vi "Beer_Pong_obstacle.vi"(8 "error in (no error)":errorcluster, 11 "Tableau lidar":dbl[][](array[numeric])=[[0.0, 1.0, 2.0, 3.0, 4.0, 5.0, 6.0, 7.0, 8.0, 9.0, 10.0, 11.0, 12.0, 13.0, 14.0, 15.0, 16.0, 17.0, 18.0, 19.0, 20.0, 21.0, 22.0, 23.0, 24.0, 25.0, 26.0, 27.0, 28.0, 29.0, 30.0, 31.0, 32.0, 33.0, 34.0, 35.0], [20.0, 15.0, 30.0, 31.0, 42.0, 50.0, 51.0, 60.0, 20.0, 15.0, 30.0, 31.0, 42.0, 50.0, 51.0, 60.0, 20.0, 15.0, 30.0, 31.0, 42.0, 50.0, 51.0, 60.0, 20.0, 15.0, 30.0, 31.0, 42.0, 50.0, 51.0, 60.0, 20.0, 15.0, 30.0, 31.0], [0.0, 0.0, 0.0, 0.0, 0.0, 0.0, 0.0, 0.0, 0.0, 0.0, 0.0, 0.0, 0.0, 0.0, 0.0, 0.0, 0.0, 0.0, 0.0, 0.0, 0.0, 0.0, 0.0, 0.0, 0.0, 0.0, 0.0, 0.0, 0.0, 0.0, 0.0, 0.0, 0.0, 0.0, 0.0, 0.0]]) -> (0 "error out":errorcluster, 2 "Distance cible":dbl, 3 "Angle cible":dbl)   [LabVIEW 2017]
panel:
  out "Cibles Detectes":dbl[][](array[numeric])
  in  "Delta Distance (cm)":dbl=10.0
  in  "Delta Angle (°)":dbl=3.0
  out "Zone 3 Bis":dbl[][](array[numeric])
  out "Detec part 3":dbl[][](array[numeric])
  out "Nbr ° à enlever début 2":i32
  out "Nbr ° à enlever fin 2":i32
  out "Début detec 3":i32
  out "Detec part 4":dbl[][](array[numeric])
  out "Moitié de Alpha":dbl
  in  "Alpha":i32=180
  in  "L3":dbl=100.0
  out "Zone 3":dbl[][](array[numeric])
  out "Zone de detection":dbl[][](array[numeric])
  out "Nbr ° à enlever fin":dbl
  out "Début detec 2":dbl
  out "Detec part 2":dbl[][](array[numeric])
  out "Nbr ° à enlever début":dbl
  out "Detec part 1":dbl[][](array[numeric])
  out "Moitié de ZM":dbl
  in  "Angle zone morte (°)":i32=170
  out "Angles / distance / statut":dbl[][](array[numeric])
  # "Face Avant"
  # "Debug"
  # "Zone morte retirée"
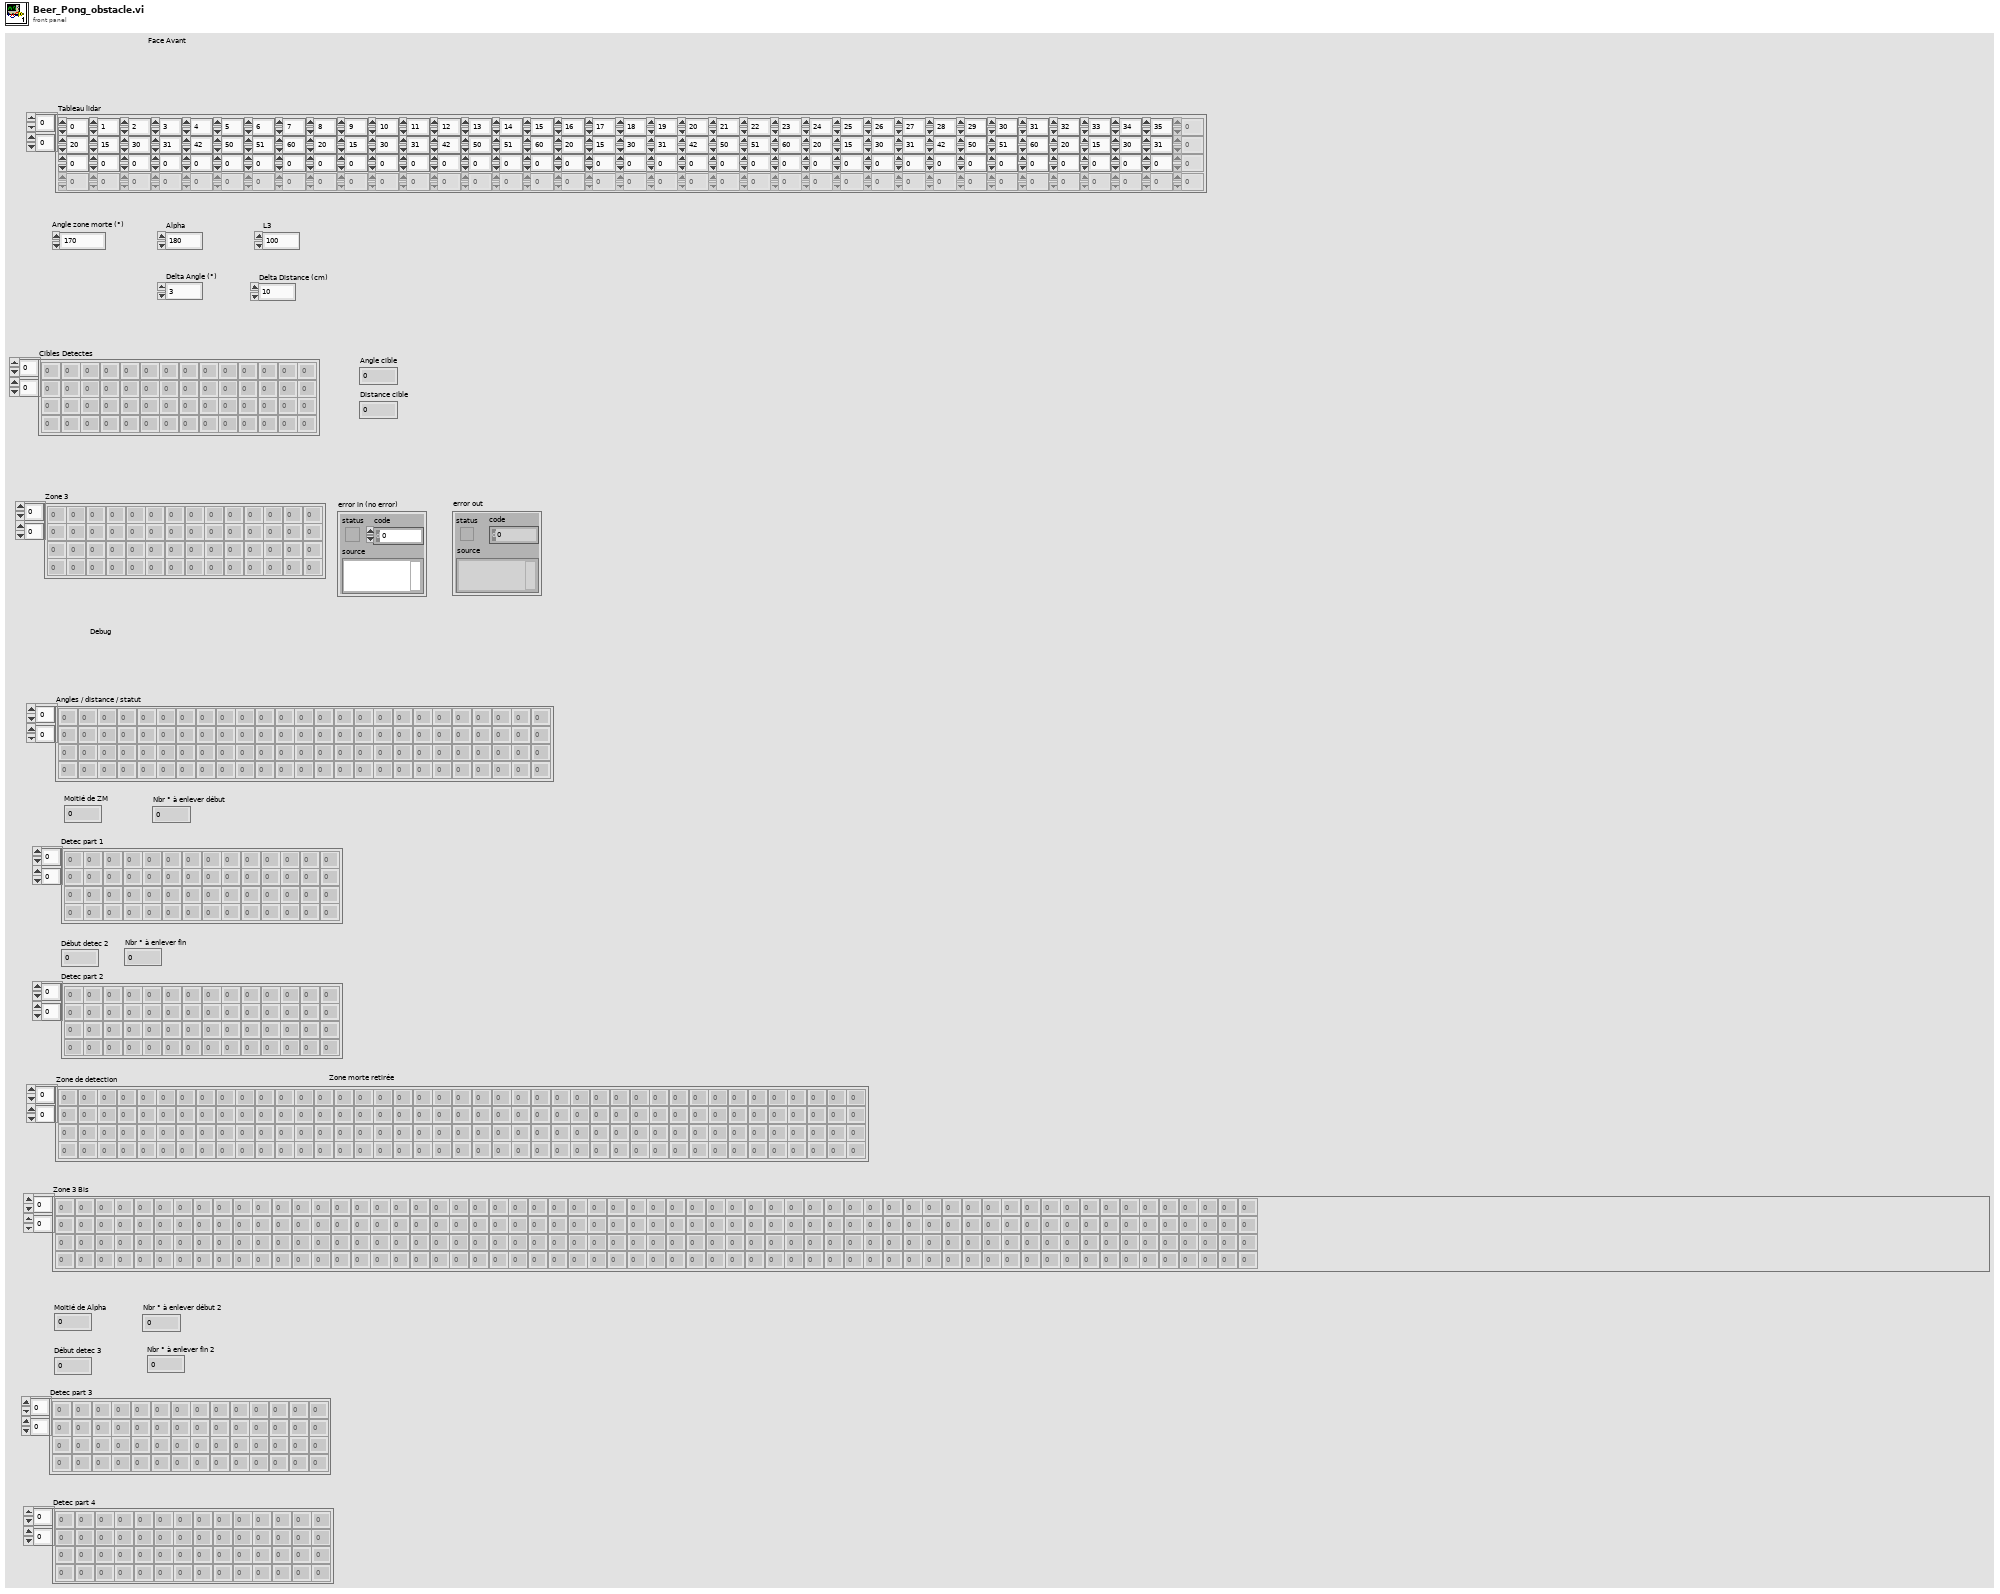
[diagram p1: front panel]
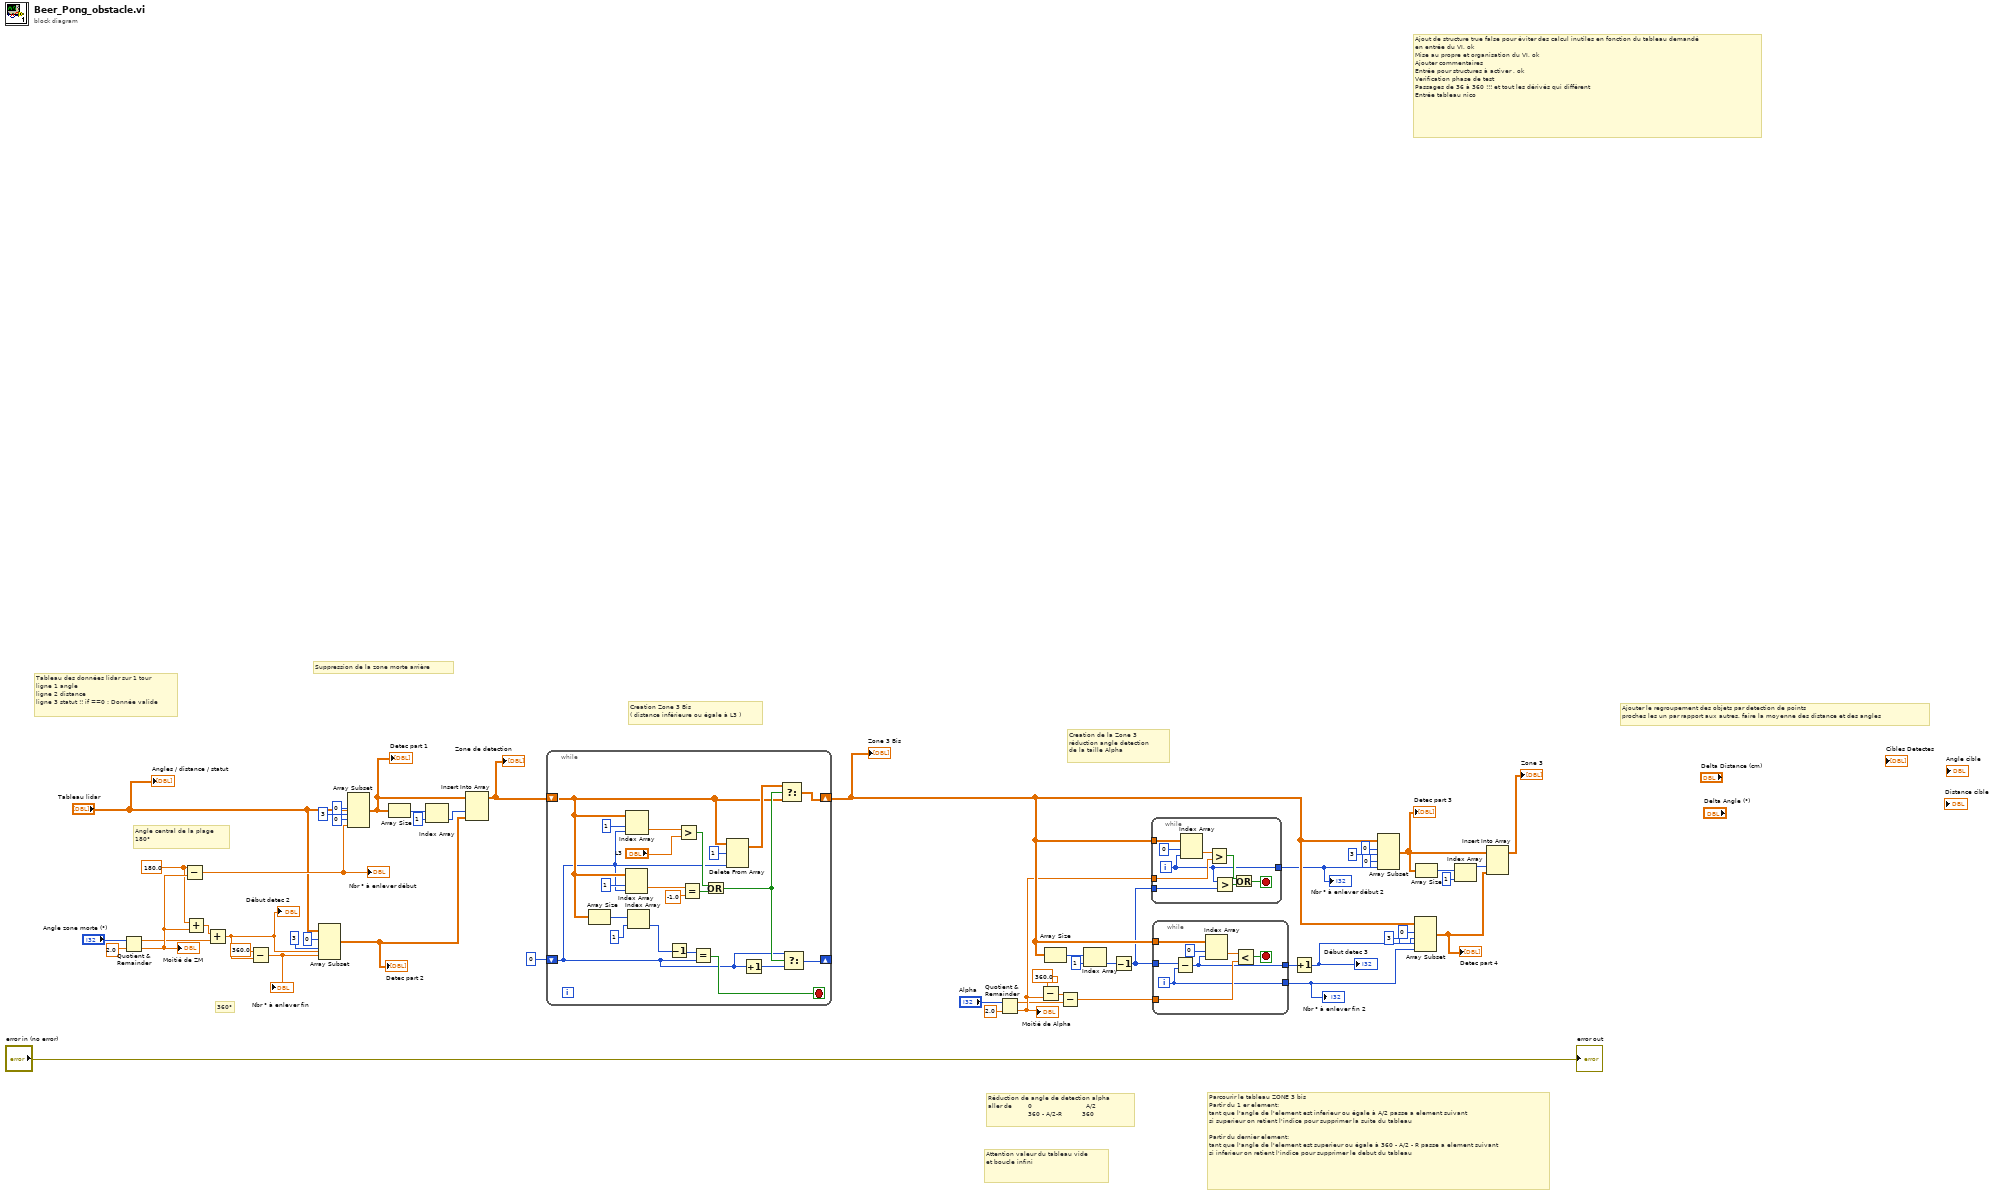
[diagram p0: block diagram]
diagram:
  w30 = 180.0 ("x")
  # "Ajouter le regroupement des objets par detection de points\nproches les un par rapport aux autres, faire la moyenne des distance et des angles"
  # "Creation de la Zone 3\nréduction angle detection \nde la taille Alpha"
  # "360°"
  # "Creation Zone 3 Bis \n( distance inférieure ou égale à L3 )"
  # "Angle central de la plage\n180°"
  # "Suppression de la zone morte arrière"
  # "Tableau des données lidar sur 1 tour\nligne 1 angle\nligne 2 distance\nligne 3 statut !! if ==0 : Donnée valide"
  # "Attention valeur du tableau vide\net boucle infini"
  # "Parcourir le tableau ZONE 3 bis\nPartir du 1 er element:\ntant que l'angle de l'element est inferieur ou égale à A/2 passe a element suivant\nsi superieur on retient l'indice pour supprimer la suite du tableau\n\nPartir du dernier element: \ntant que l'angle de l'element est superieur ou égale à 360 - A/2 - R passe a element suivant\nsi inferieur on retient l'indice pour supprimer le debut du tableau"
  # "Réduction de angle de detection alpha\naller de        0                           A/2\n                    360 - A/2-R          360"
  # "Ajout de structure true false pour éviter des calcul inutiles en fonction du tableau demandé \nen entrée du VI, ok\nMise au propre et organisation du VI, ok\nAjouter commentaires\nEntrée pour structures à activer , ok\nVerification phase de test\nPassages de 36 à 360 !!! et tout les dérivés qui différent\nEntrée tableau nico"
  n1 = Quotient & Remainder(x="Angle zone morte (°)", y=2.0) -> (x-y*floor(x/y)=w39:dbl, floor(x/y)=w48:dbl)
  "Moitié de ZM" <- w48
  n2 = Subtract(x=w30, y=w48) -> (x-y=w29:dbl)
  "Nbr ° à enlever début" <- w29
  n3 = Add(x=w30, y=w48) -> (x+y=w40:dbl)
  n4 = Add(x=w40, y=w39) -> (x+y=w33:dbl)
  "Début detec 2" <- w33
  n5 = Subtract(x=360.0, y=w33) -> (x-y=w46:dbl)
  "Nbr ° à enlever fin" <- w46
  n6 = Array Subset(array="Tableau lidar", index (row)=0 ("index"), length (row)=3 ("length"), index (col)=w33, length (col)=w46) -> (w35:dbl[][])
  "Detec part 2" <- w35
  n7 = Array Subset(array="Tableau lidar", index (row)=0 ("index"), length (row)=3 ("length"), index (col)=0 ("index"), length (col)=w29) -> (w36:dbl[][])
  "Detec part 1" <- w36
  n8 = Array Size(array=w36) -> (size(s)=w38:i32[])
  n9 = Index Array(array=w38, index=1) -> (element=w34:i32)
  n10 = Insert Into Array(array=w36, index (col)=w34, new element=w35) -> (w31:dbl[][])  [unwired: 1 in]
  "Zone de detection" <- w31
  n11 = while {
    shift-right: [w64] -> w28
    shift-left: w31 -> [w54]
    shift-right: [w66] -> _
    shift-left: 0 -> [w53]
    stop <- w63 stop-if-true
    n12 = Array Size(array=w54) -> (size(s)=w68:i32[])
    n13 = Index Array(array=w54, index (row)=1 ("disabled index (row)"), index (col)=w53) -> (element=w52:dbl)
    n14 = Index Array(array=w54, index (row)=1 ("disabled index (row)"), index (col)=w53) -> (element=w70:dbl)
    n15 = Index Array(array=w68, index=1) -> (element=w61:i32)
    n16 = Decrement(x=w61) -> (x-1=w62:i32)
    n17 = Greater?(x=w70, y="L3") -> (0:w57:bool)
    n18 = Equal?(x=w52, y=-1.0) -> (x = y?=w58:bool)
    n19 = Equal?(x=w62, y=w53) -> (x = y?=w63:bool)
    n20 = Or(x=w57, y=w58) -> (x .or. y?=w59:bool)
    n21 = Delete From Array(array=w54, length=1, index (col)=w53) -> (array with subset deleted=w69:dbl[][])  [unwired: 1 in, 1 out]
    n22 = Increment(x=w53) -> (x+1=w65:i32)
    n23 = Select(t=w69, s=w59, f=w54) -> (s? t:f=w64:dbl[][])
    n24 = Select(t=w53, s=w59, f=w65) -> (s? t:f=w66:i32)
  }
  "Zone 3 Bis" <- w28
  n25 = Quotient & Remainder(x="Alpha", y=2.0) -> (x-y*floor(x/y)=w12:dbl, floor(x/y)=w26:dbl)
  "Moitié de Alpha" <- w26
  n26 = Subtract(x=360.0, y=w26) -> (x-y=w11:dbl)
  n27 = Array Size(array=w28) -> (size(s)=w13:i32[])
  n28 = Subtract(x=w11, y=w12) -> (x-y=w15:dbl)
  n29 = Index Array(array=w13, index=1) -> (element=w14:i32)
  n30 = Decrement(x=w14) -> (x-1=w19:i32)
  n31 = while {
    tunnel: w28 -> [w81]
    tunnel: w26 -> [w79]
    tunnel: [w74] -> w22
    tunnel: w19 -> [w73]
    i -> [w74]
    stop <- w76 stop-if-true
    n32 = Index Array(array=w81, index (row)=0, index (col)=w74) -> (element=w78:dbl)
    n33 = Greater?(x=w78, y=w79) -> (0:w77:bool)
    n34 = Greater?(x=w74, y=w73) -> (0:w75:bool)
    n35 = Or(x=w77, y=w75) -> (x .or. y?=w76:bool)
  }
  "Nbr ° à enlever début 2" <- w22
  n36 = while {
    tunnel: w28 -> [w88]
    tunnel: w19 -> [w87]
    tunnel: w15 -> [w85]
    tunnel: [w84] -> w16
    tunnel: [w83] -> w23
    i -> [w83]
    stop <- w82 stop-if-true
    n37 = Subtract(x=w87, y=w83) -> (x-y=w84:i32)
    n38 = Index Array(array=w88, index (row)=0, index (col)=w84) -> (element=w86:dbl)
    n39 = Less?(x=w86, y=w85) -> (x < y?=w82:bool)
  }
  "Nbr ° à enlever fin 2" <- w23
  n40 = Increment(x=w16) -> (x+1=w24:i32)
  "Début detec 3" <- w24
  n41 = Array Subset(array=w28, index (row)=0 ("index"), length (row)=3 ("length"), index (col)=0 ("index"), length (col)=w22) -> (w20:dbl[][])
  "Detec part 3" <- w20
  n42 = Array Subset(array=w28, index (row)=0 ("index"), length (row)=3 ("length"), index (col)=w24, length (col)=w23) -> (w21:dbl[][])
  "Detec part 4" <- w21
  n43 = Array Size(array=w20) -> (size(s)=w17:i32[])
  n44 = Index Array(array=w17, index=1) -> (element=w18:i32)
  n45 = Insert Into Array(array=w20, index (col)=w18, new element=w21) -> (→"Zone 3":dbl[][])  [unwired: 1 in]
  "error out" <- "error in (no error)"
  "Angles / distance / statut" <- "Tableau lidar"
